vi "SetValueByArrayName.vi"(0 "VI Reference In":refnum<vi>, 2 "delimiter (>>)":string=">>", 5 "Control Path":string, 7 "Name Array":T1[](array[typedef]), 11 "Error In":errorcluster) -> (4 "VI Reference Out":refnum<vi>, 15 "Error Out":errorcluster)   [LabVIEW 2016, in "Drona.lvlib" / "ControlValue.lvlib" / "StimulusMCListbox.lvlib"]
doc: "Sets value(signaling) for the multi select multi column listbox control whose first column item names with its occurrence are specified. Set the value as 1 in occurrence to select the first occurrence of an item. \n\nThe input control name is given as a string , incase of path, use delimiters inbetween the path."
uses:
  StimulusMCListbox.lvlib
  typedef/Name&Occurrence.ctl
  <userlib>/_OpenG.lib/array/array.llb/Search 1D Array (String)__ogtk.vi
  <vilib>/Utility/error.llb/Error Cluster From Error Code.vi
  <vilib>/ErrorRing/Error Ring.xnode
  Drona.lvlib
  Get/GetControlRef/GetControlRef.lvlib
  ControlValue.lvlib
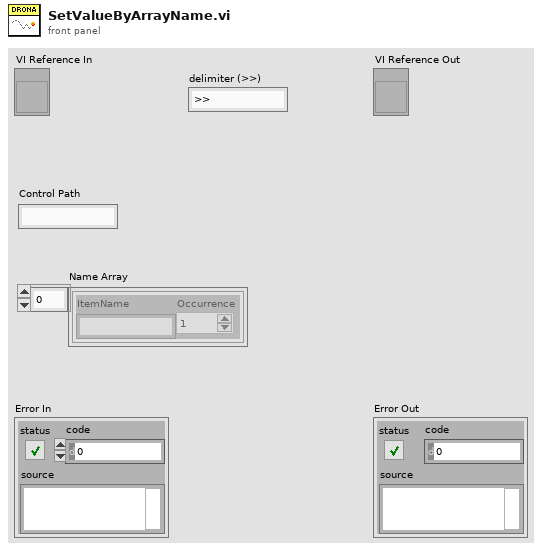
[diagram p1: front panel]
types:
  T1 = typedef "Drona.lvlib/ControlValue.lvlib/Name&Occurrence.ctl" = cluster{"ItemName":string, "Occurrence":i32}
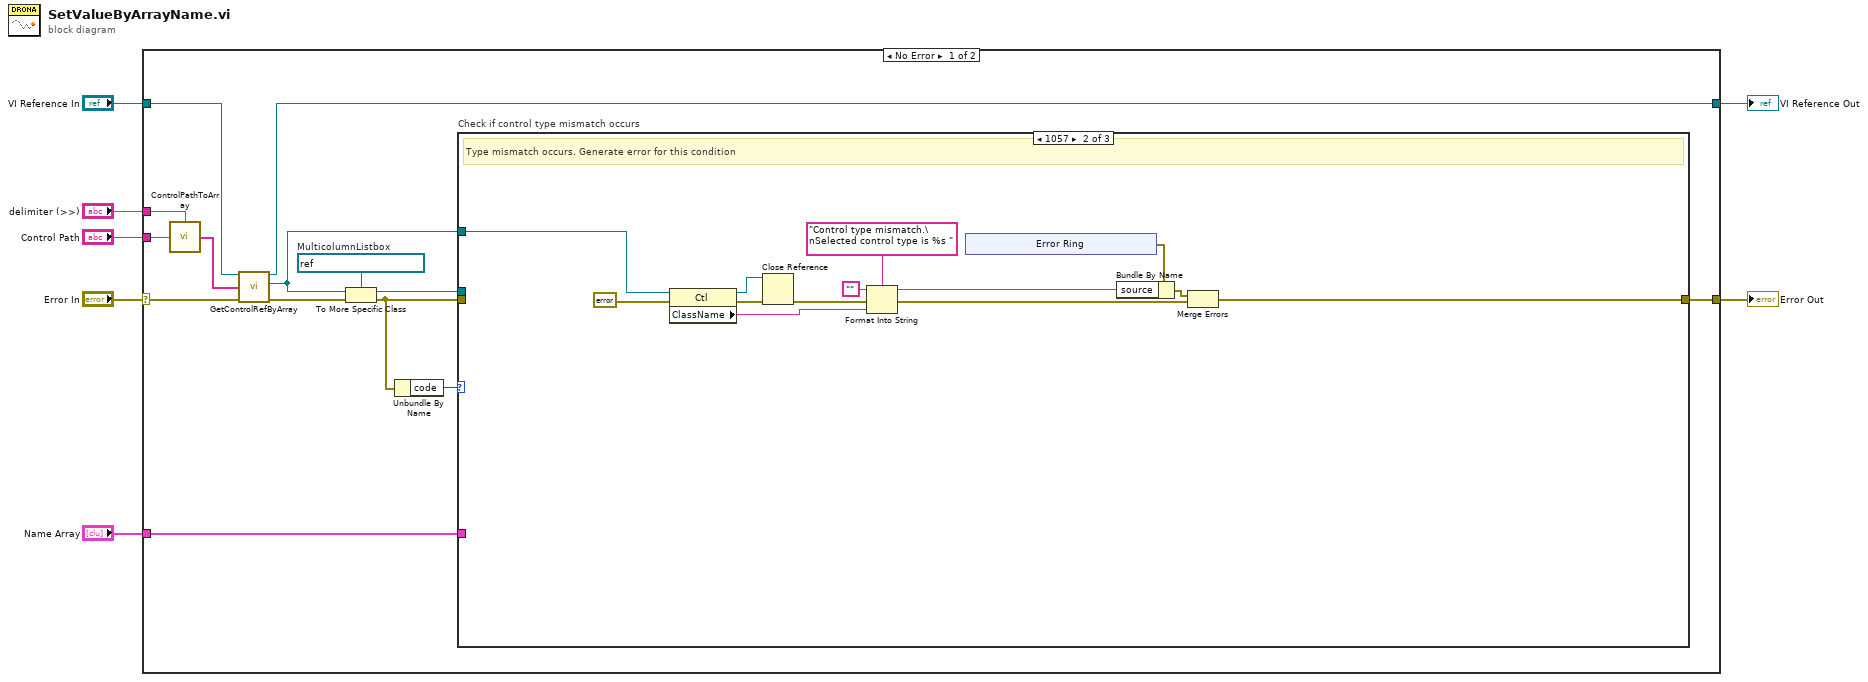
[diagram p0: block diagram]
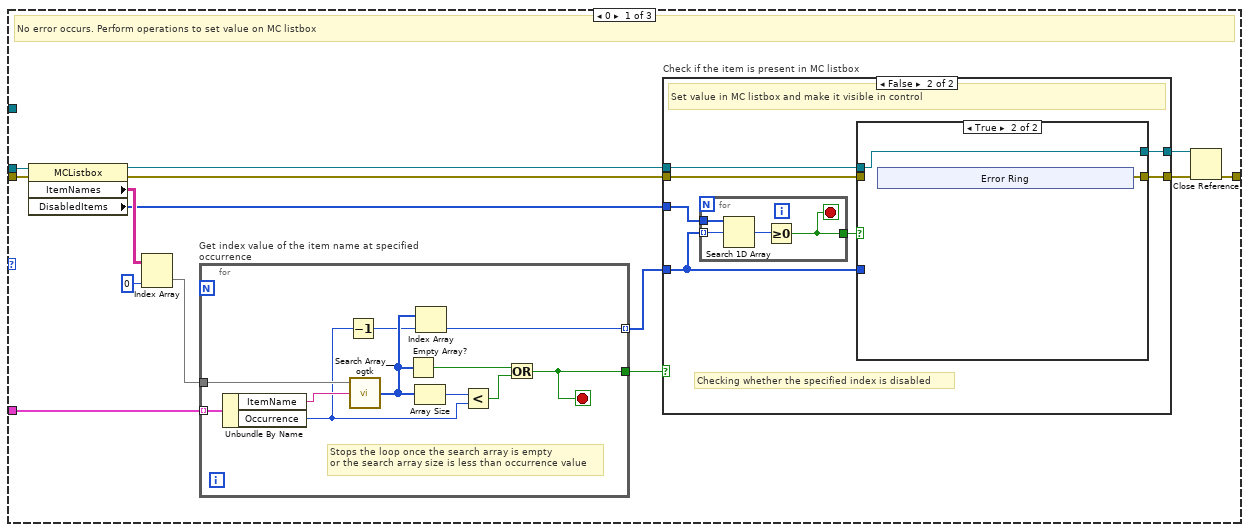
[diagram p2: hidden frame]
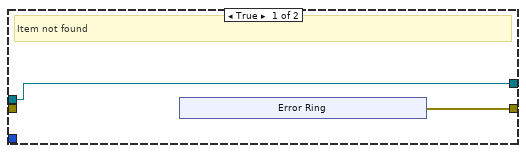
[diagram p3: hidden frame]
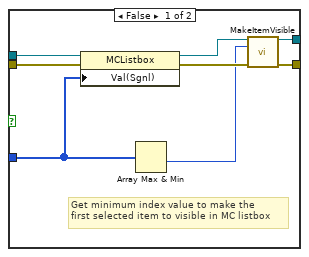
[diagram p4: hidden frame]
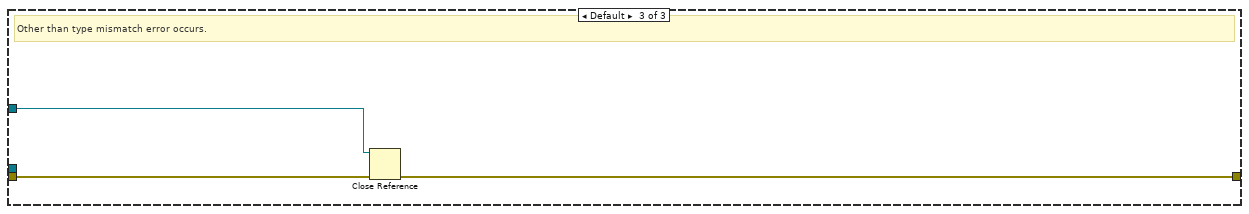
[diagram p5: hidden frame]
diagram:
  n1 = case shown="No Error" "Error In" {
    selector: "Error In" -> [w16 w102]
    tunnel: [w17 w102] -> w6
    tunnel: "VI Reference In" -> [w15 w101]
    tunnel: "Control Path" -> [w19 _]
    tunnel: [w12 w101] -> w3
    tunnel: "delimiter (>>)" -> [w18 _]
    tunnel: "Name Array" -> [w11 _]
    frame No Error {
      w21 = refnum<vi> refnum  # MulticolumnListbox
      n2 = call "ControlPathToArray.vi"("Control Name"=w19, "delimiter (>>)"=w18) -> ("Control Path"=w14:string[])
      n3 = call "GetControlRefByArray.vi"("VI Reference In"=w15, "Control Path"=w14, "error In"=w16) -> ("VI Reference Out"=w12:refnum<vi>, "Ctl Refnum"=w8:refnum<vi>, "error out"=w13:errorcluster)  [unwired: 10 in]
      n4 = To More Specific Class(target class=w21, reference=w8, error in=w13) -> (specific class reference=w20:refnum<vi>, error out=w10:errorcluster)
      n5 = Unbundle By Name(w10) -> ("code"=w9:i32)
      n6 = case "Check if control type mismatch occurs" shown="1057" w9 {
        tunnel: w10 -> [w35 _ w100]
        tunnel: w20 -> [w34 _ _]
        tunnel: [w33 w80 w99] -> w17
        tunnel: w11 -> [w30 _ _]
        tunnel: w8 -> [_ w81 w98]
        frame 0 {
          # "No error occurs. Perform operations to set value on MC listbox"
          n7 = property class="MCListbox"(reference=w34, error in=w35) -> (reference out=w28:refnum<vi>, error out=w29:errorcluster, "ItemNames"=w25:string[][], "DisabledItems"=w22:i32[])
          n8 = Index Array(array=w25, index (col)=0 ("disabled index (col)")) -> (element=w23:string[])  [unwired: 1 in]
          n9 = for "Get index value of the item name at specified occurrence" {
            tunnel: w23 -> [w45]
            tunnel: w30 -> [w46] mode=indexing
            tunnel: [w37] -> w27 mode=indexing
            tunnel: [w36] -> w26
            stop <- w36 stop-if-true
            # "Stops the loop once the search array is empty \nor the search array size is less than occurrence value"
            n10 = Unbundle By Name(w46) -> ("ItemName"=w44:string, "Occurrence"=w39:i32)
            n11 = Decrement(x=w39) -> (x-1=w38:i32)
            n12 = call-poly <userlib>:"Search Array__ogtk.vi"("Array"=w45, "Element Data"=w44) -> ("Indices of Elements"=w40:i32[])  [unwired: 7 in]
            n13 = Empty Array?(array=w40) -> (empty?=w41:bool)
            n14 = Array Size(array=w40) -> (size(s)=w43:i32)
            n15 = Index Array(array=w40, index=w38) -> (element=w37:i32)
            n16 = Less?(x=w43, y=w39) -> (x < y?=w42:bool)
            n17 = Or(x=w41, y=w42) -> (x .or. y?=w36:bool)
          }
          n18 = case "Check if the item is present in MC listbox" shown="False" w26 {
            tunnel: [w48 w60] -> w32
            tunnel: [w47 w59] -> w31
            tunnel: w29 -> [_ w58]
            tunnel: w28 -> [w47 w57]
            tunnel: w27 -> [_ w55]
            tunnel: w22 -> [_ w56]
            frame True {
              # "Item not found"
              n19 = xnode "Error Ring"() -> ("error out"=w48:errorcluster)
            }
            frame False {
              # "Checking whether the specified index is disabled"
              # "Set value in MC listbox and make it visible in control"
              n20 = for {
                tunnel: w55 -> [w64] mode=indexing
                tunnel: [w61] -> w54
                tunnel: w56 -> [w62]
                stop <- w61 stop-if-true
                n21 = Search 1D Array(1D array=w62, element=w64) -> (index of element=w63:i32)  [unwired: 1 in]
                n22 = Greater Or Equal To 0?(x=w63) -> (x >= 0?=w61:bool)
              }
              n23 = case shown="True" w54 {
                tunnel: [w71 w73] -> w60
                tunnel: [w69 w74] -> w59
                tunnel: w58 -> [w67 _]
                tunnel: w57 -> [w66 w74]
                tunnel: w55 -> [w65 _]
                frame False {
                  # "Get minimum index value to make the \nfirst selected item to visible in MC listbox"
                  n24 = property class="MCListbox"(reference=w66, error in=w67, "Val(Sgnl)"=w65) -> (reference out=w70:refnum<vi>, error out=w72:errorcluster)
                  n25 = Array Max & Min(array=w65) -> (min value=w68:i32)  [unwired: 3 out]
                  n26 = call "MakeItemVisible.vi"("MC ListBox Ref In"=w70, "Item Index"=w68, "Error In"=w72) -> ("MC ListBox Ref Out"=w69:refnum<vi>, "Error Out"=w71:errorcluster)  [unwired: 11 in]
                }
                frame True {
                  n27 = xnode "Error Ring"() -> ("error out"=w73:errorcluster)
                }
              }
            }
          }
          n28 = Close Reference(reference=w31, error in (no error)=w32) -> (error out=w33:errorcluster)
        }
        frame 1057 {
          # "Type mismatch occurs. Generate error for this condition"
          n29 = property class="Ctl"(reference=w81, error in=errorcluster {"status"=FALSE, "code"=0, "source"=""} ("error out")) -> (reference out=w82:refnum<vi>, error out=w92:errorcluster, "ClassName"=w89:string)
          n30 = Close Reference(reference=w82, error in (no error)=w92) -> (error out=w83:errorcluster)
          n31 = Format Into String(format string="Control type mismatch.\nSelected control type is %s ", initial string="", error in=w83, w89) -> (resulting string=w86:string, error out=w84:errorcluster)
          n32 = xnode "Error Ring"() -> ("error out"=w87:errorcluster)
          n33 = Bundle By Name(cluster=w87, "source"=w86) -> (w85:errorcluster)
          n34 = Merge Errors(w85, w84) -> (w80:errorcluster)
        }
        frame Default {
          # "Other than type mismatch error occurs."
          n35 = Close Reference(reference=w98, error in (no error)=w100) -> (error out=w99:errorcluster)
        }
      }
    }
    frame Error {
    }
  }
  "Error Out" <- w6
  "VI Reference Out" <- w3
